vi "Get .Net Container.vi"(11 "SourceGrid in":refnum<class "SourceGrid.lvclass">) -> (2 ".NET Container":refnum<k24>, 3 "SourceGrid out":refnum<class "SourceGrid.lvclass">)   [LabVIEW 2020, in "SourceGrid.lvlib" / "SourceGrid.lvclass"]
uses:
  SourceGrid.lvclass
  D:/git/Sourcegrid-LabVIEW/source/SourceGrid.dll
  SourceGrid.dll
  SourceGrid.lvclass/SourceGrid.ctl
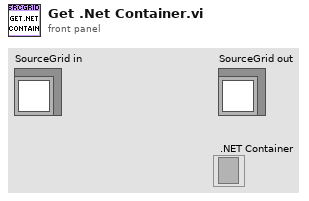
[diagram p1: front panel]
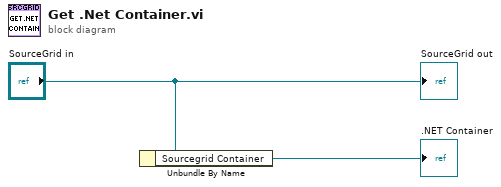
[diagram p0: block diagram]
diagram:
  n1 = Unbundle By Name("SourceGrid in") -> ("Sourcegrid Container"=→".NET Container":refnum<k24>)
  "SourceGrid out" <- "SourceGrid in"
